vi "FRC Wizard - Robot.vi"() -> ()   [LabVIEW 2023]
uses:
  <resource>/plugins/NewDialogFiles/ProjectWizards/ProjectWizard.llb/ProjectWizard Navigation Button States.ctl
  <resource>/plugins/NewDialogFiles/ProjectWizards/ProjectWizard.llb/ProjectWizard Navigation Button State.ctl
  <resource>/plugins/NewDialogFiles/ProjectWizards/ProjectWizard.llb/ProjectWizard Navigation Buttons.ctl
  <resource>/plugins/NewDialogFiles/ProjectWizards/FRC/FRC Strings.vi
  <resource>/plugins/NewDialogFiles/ProjectWizards/FRC/frc project type.ctl
panel:
  out "project folder flag":bool
  in  "Tab Control":enum32{"Page 1"}(tab)
  in  "Framework Choice":enum32{"Robot Project"}(radio)
  in  "Team number":string="xxyy"
  out "Picture-0":picture
  in  "Project folder":path
  in  "Project name":string
  in  "Shutdown user event":refnum<user-event>
  in  "Subpanel Path user event":refnum<user-event>
  in  "Window Title user event":refnum<user-event>
  in  "Navigation Button States user event":refnum<user-event>
  in  "Navigation Buttons user event":refnum<event-registration>
  # "Select project name, folder"
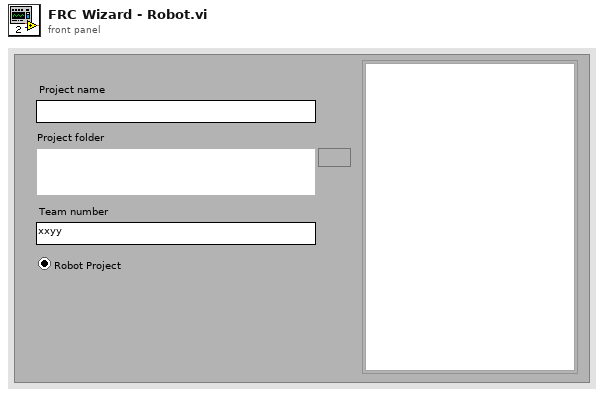
[diagram p1: front panel]
types:
  T1 = enum16{"Display", "Configure", "Hide Dialog", "Discard Ref"}
  T2 = typedef "ProjectWizard Navigation Button States.ctl" = T3[]
  T3 = typedef "ProjectWizard Navigation Button State.ctl" = cluster{"Navigation Button":T4, "Disabled":u8}
  T4 = typedef "ProjectWizard Navigation Buttons.ctl" = enum16{"Back", "Next", "Finish", "Cancel", "Help"}
  T5 = typedef "frc project type.ctl" = enum16{"arcade", "command control", "maze", "ball shooter", "dashboard", "dashboard simple", "dashboard maze", "dashboard shooter", "romi", "XRP"}
  T6 = typedef "RTNPA Navigation Buttons.ctl" = enum16{"Back", "Next", "Finish", "Cancel", "Help"}
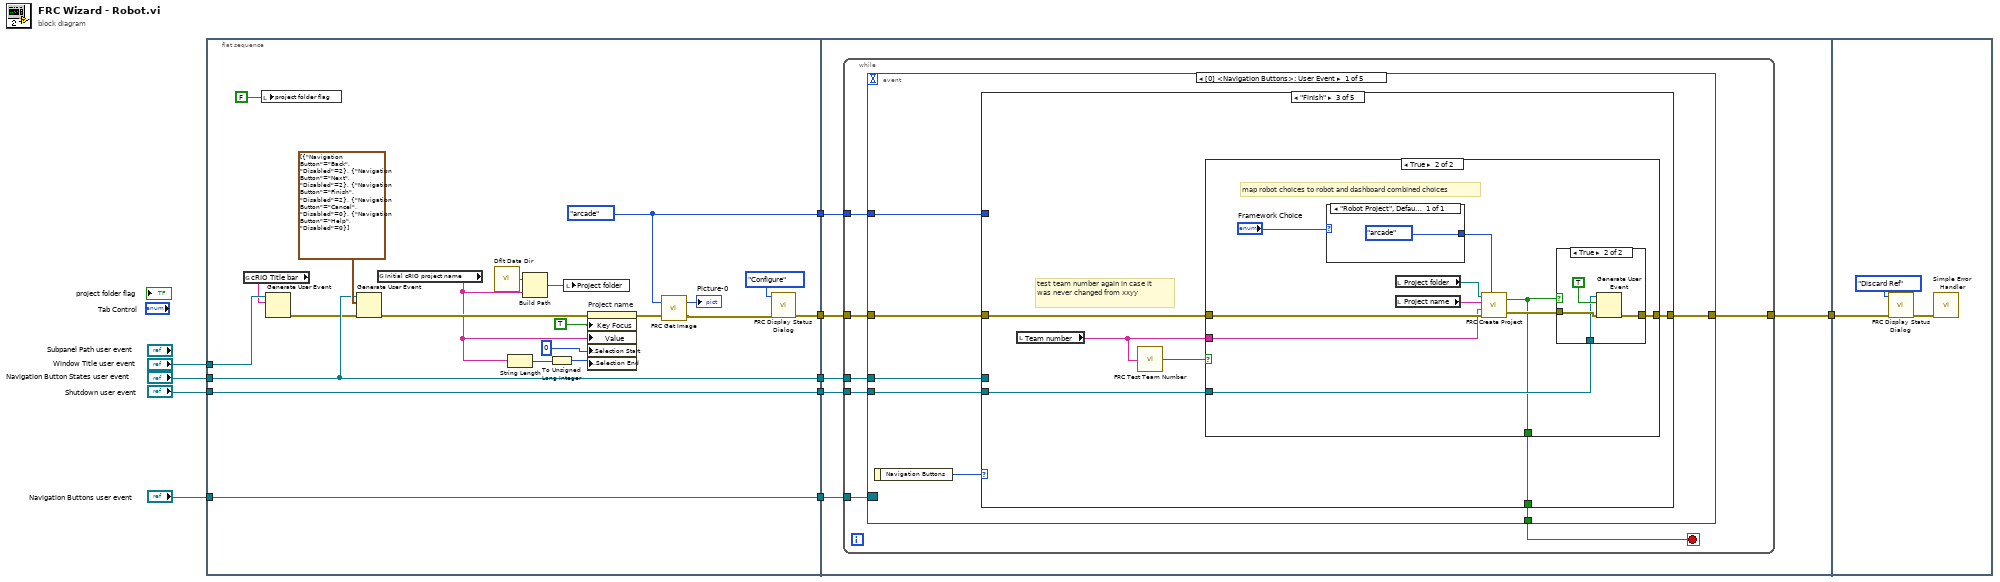
[diagram p0: block diagram]
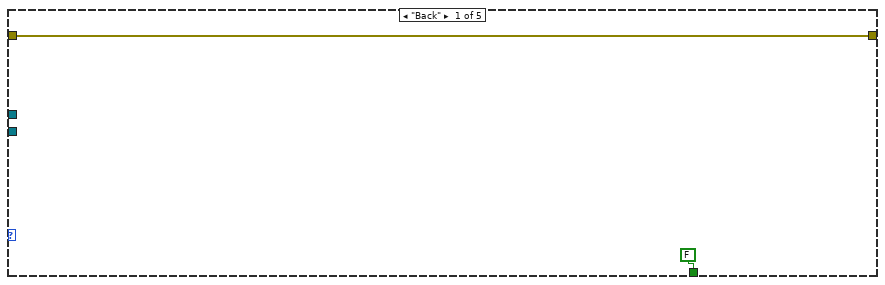
[diagram p2: hidden frame]
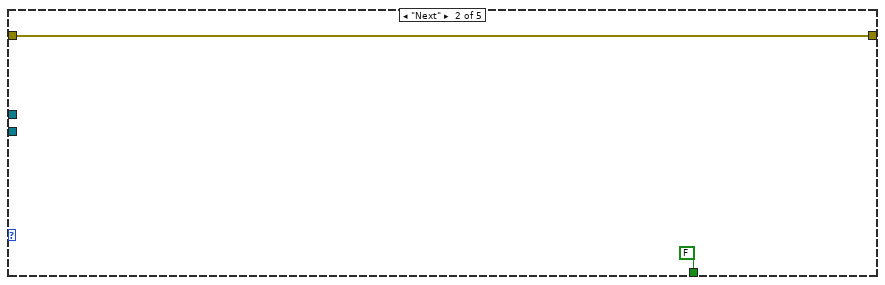
[diagram p3: hidden frame]
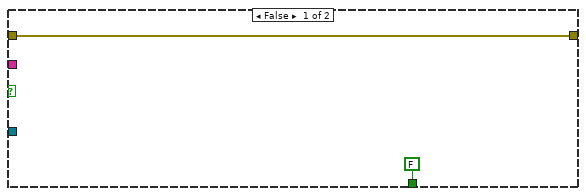
[diagram p4: hidden frame]
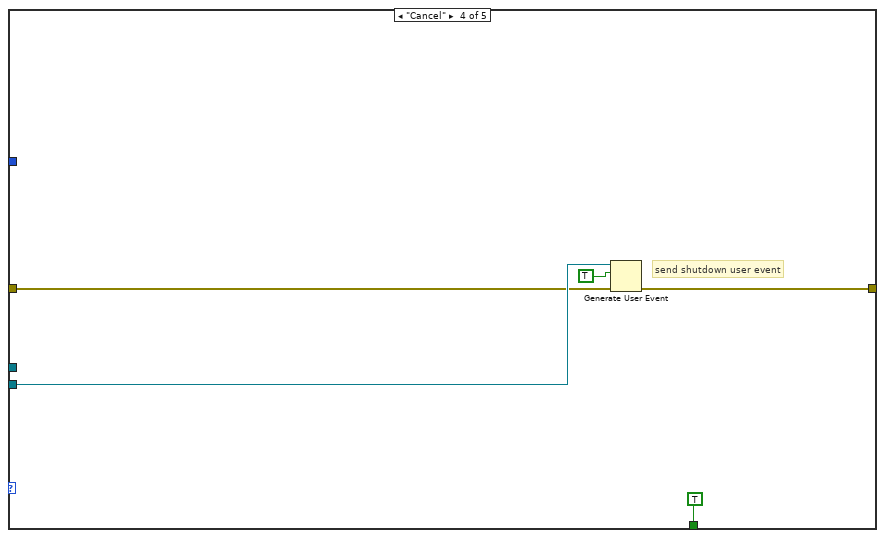
[diagram p6: hidden frame]
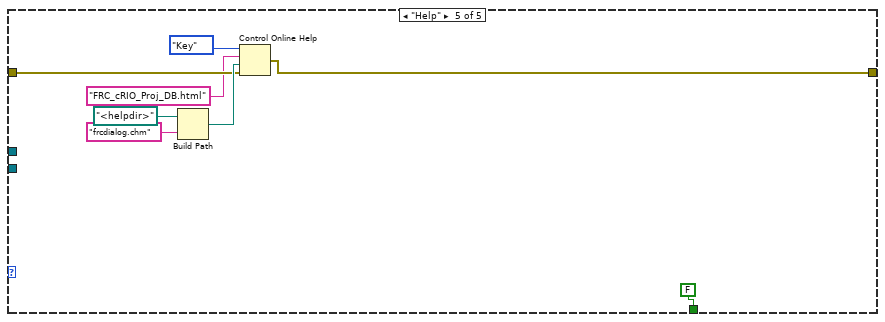
[diagram p7: hidden frame]
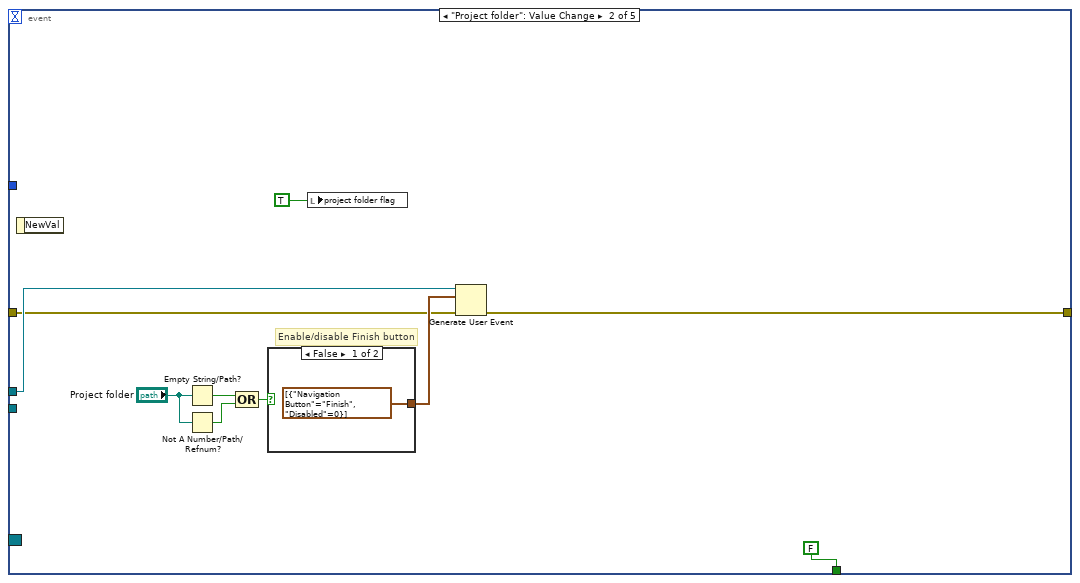
[diagram p8: hidden frame]
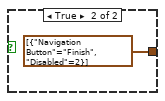
[diagram p9: hidden frame]
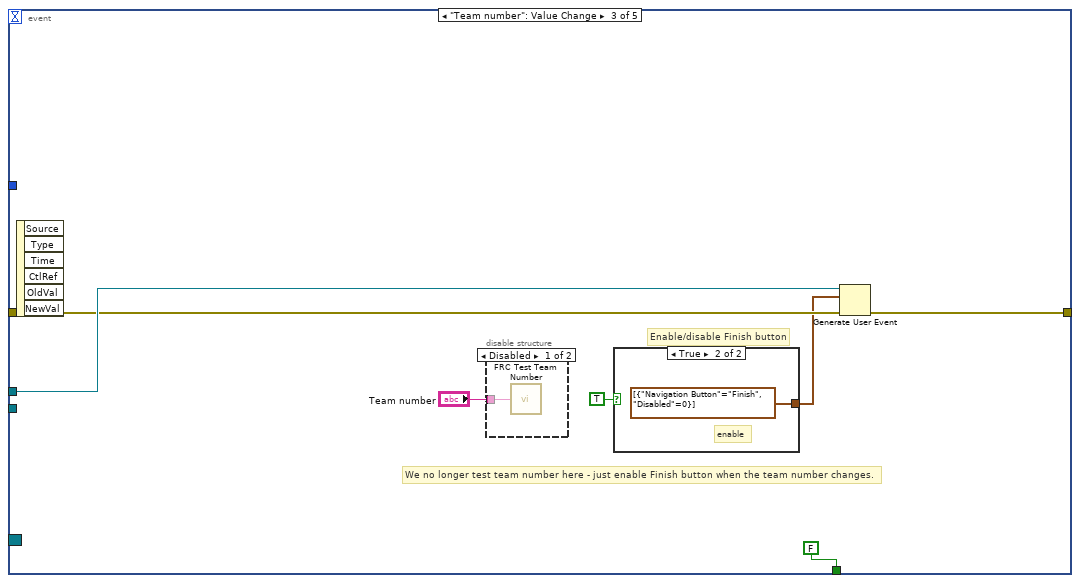
[diagram p10: hidden frame]
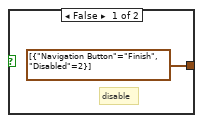
[diagram p12: hidden frame]
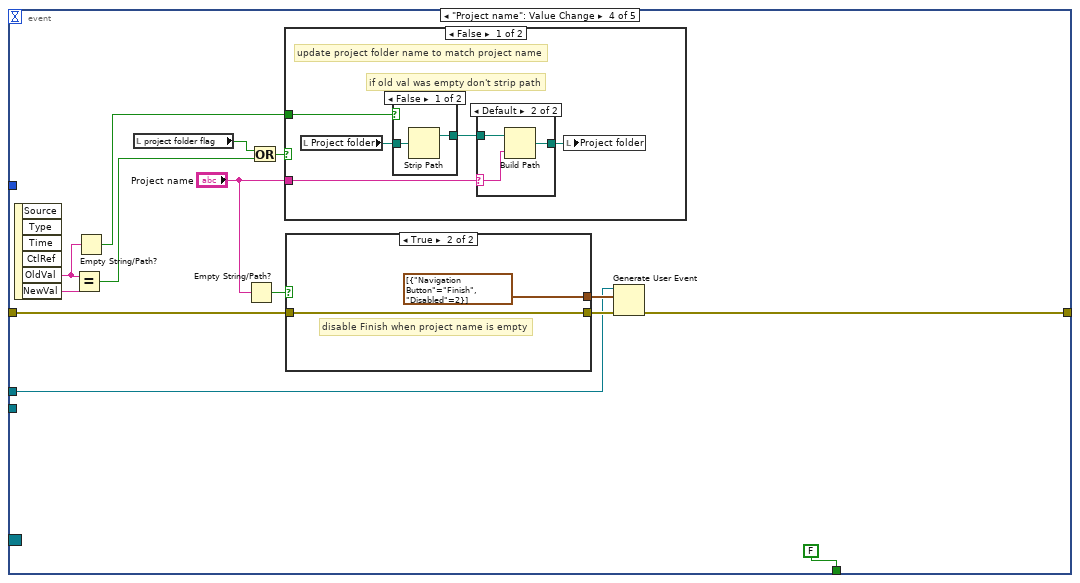
[diagram p13: hidden frame]
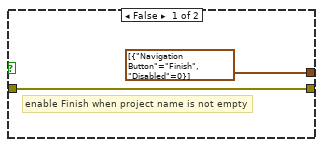
[diagram p17: hidden frame]
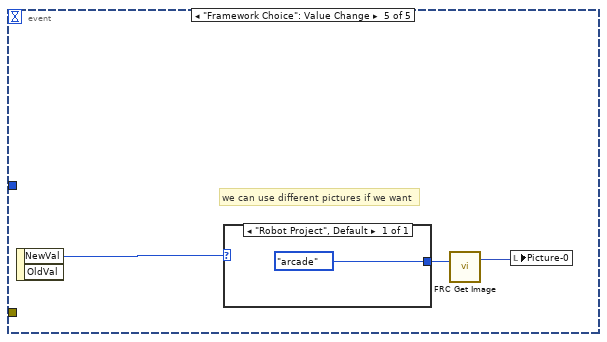
[diagram p18: hidden frame]
diagram:
  n1 = flat-sequence {
    tunnel: [w22] -> w6
    tunnel: [w32] -> w5
    tunnel: [w31] -> w4
    tunnel: [w18] -> w3
    tunnel: "Navigation Button States user event" -> [w22]
    tunnel: "Window Title user event" -> [w29]
    tunnel: "Navigation Buttons user event" -> [w32]
    tunnel: "Shutdown user event" -> [w31]
    tunnel: [w11] -> w1
    tunnel: w6 -> [w38]
    tunnel: w5 -> [w37]
    tunnel: w4 -> [w35]
    tunnel: w3 -> [w34]
    tunnel: [w36] -> w2
    tunnel: w1 -> [w33]
    tunnel: w2 -> [w151]
    frame #0 {
      w11 = frc_project_type."arcade" ("frc project type")
      n2 = global read "FRC Strings.vi" "cRIO Title bar"() -> (w26:string)
      n3 = local write "project folder flag"(FALSE ("project folder flag")) -> ()
      n4 = Generate User Event(user event=w29, event data cluster=w26) -> (error out=w21:errorcluster)  [unwired: 2 in, 1 out]
      n5 = Generate User Event(user event=w22, event data cluster=T2 [{"Navigation Button"=enum."Back", "Disabled"=2}, {"Navigation Button"=enum."Next", "Disabled"=2}, {"Navigation Button"=enum."Finish", "Disabled"=2}, {"Navigation Button"=enum."Cancel", "Disabled"=0}, {"Navigation Button"=enum."Help", "Disabled"=0}] ("Navigation Button States"), error in=w21) -> (error out=w19:errorcluster)  [unwired: 1 in, 1 out]
      n6 = global read "FRC Strings.vi" "Initial cRIO project name"() -> (w15:string)
      n7 = call <vilib>:"Dflt Data Dir.vi"() -> ("App:Default Data Directory"=w27:path)
      n8 = String Length(string=w15) -> (length=w23:i32)
      n9 = Build Path(base path=w27, name or relative path=w15) -> (appended path=w20:path)
      n10 = To Unsigned Long Integer(number=w23) -> (unsigned 32bit integer=w24:u32)
      n11 = local write "Project folder"(w20) -> ()
      n12 = property on="Project name" class="Str"(error in=w19, "Key Focus"=TRUE, "Value"=w15, "Text.Selection Start"=u32 0 ("Text.Selection:Start"), "Text.Selection End"=w24) -> (error out=w14:errorcluster)  [unwired: 1 in, 1 out]
      n13 = call <resource>:"FRC Get Image.vi"("error in"=w14, "frc project type"=w11) -> ("error out"=w13:errorcluster, "new picture"=→"Picture-0":picture)
      n14 = call <resource>:"FRC Display Status Dialog.vi"("error in"=w13, "Mode"=T1."Configure") -> ("error out"=w18:errorcluster)  [unwired: 2 in, 7 out]
    }
    frame #1 {
      n15 = while {
        tunnel: w37 -> [w45]
        tunnel: w38 -> [w44]
        tunnel: w34 -> [w43]
        tunnel: [w41] -> w36
        tunnel: w35 -> [w40]
        tunnel: w33 -> [w39]
        stop <- w42 stop-if-true
        n16 = event shown="[0] <Navigation Buttons>: User Event" {
          selector: w45 -> [_ _ _ _ _]
          dyn-events: _ -> [_ _ _ _ _]
          timeout: _ -> [_ _ _ _ _]
          tunnel: w44 -> [w48 w98 w111 w123 _]
          tunnel: w43 -> [w50 w97 w110 w128 _]
          tunnel: [w51 FALSE ("x = y?") FALSE ("x = y?") FALSE ("x = y?") _] -> w42
          tunnel: [w49 w99 w112 w125 _] -> w41
          tunnel: w40 -> [w47 _ _ _ _]
          tunnel: w39 -> [w46 _ _ _ _]
          event User Event {
            n17 = event-data() -> ("Navigation Buttons"=w52:T6)  [unwired: 1 out]
            n18 = case shown="\"Finish\"" w52 {
              tunnel: [FALSE ("x = y?") FALSE w59 TRUE FALSE] -> w51
              tunnel: w50 -> [w53 w55 w61 w81 w88]
              tunnel: [w53 w55 w62 w82 w89] -> w49
              tunnel: w48 -> [_ _ _ _ _]
              tunnel: w47 -> [_ _ w60 w83 _]
              tunnel: w46 -> [_ _ _ _ _]
              frame "Back" {
              }
              frame "Next" {
              }
              frame "Finish" {
                # "test team number again in case it was never changed from xxyy"
                n19 = local read "Team number"() -> (w58:string)
                n20 = call <resource>:"FRC Test Team Number.vi"("Team number"=w58) -> ("pass?"=w57:bool)  [unwired: 14 in]
                n21 = case shown="True" w57 {
                  tunnel: [w63 w74] -> w62
                  tunnel: w61 -> [w63 w72]
                  tunnel: w60 -> [_ w71]
                  tunnel: [FALSE ("proceed?") w68] -> w59
                  tunnel: w58 -> [_ w65]
                  frame False {
                  }
                  frame True {
                    # "map robot choices to robot and dashboard combined choices"
                    n22 = case shown="\"Robot Project\", Default" "Framework Choice" {
                      tunnel: [frc_project_type."arcade" ("frc project type")] -> w66
                      frame "Robot Project", Default {
                      }
                    }
                    n23 = local read "Project folder"() -> (w69:path)
                    n24 = local read "Project name"() -> (w70:string)
                    n25 = call <resource>:"FRC Create Project.vi"("Project folder"=w69, "Project name"=w70, "Team number"=w65, "error in"=w72, "frc project type"=w66) -> ("proceed?"=w68:bool, "error out"=w73:errorcluster)
                    n26 = case shown="True" w68 {
                      tunnel: [w76 w80] -> w74
                      tunnel: w73 -> [w76 w78]
                      tunnel: w71 -> [_ w77]
                      frame False {
                      }
                      frame True {
                        n27 = Generate User Event(user event=w77, event data cluster=TRUE ("event data"), error in=w78) -> (error out=w80:errorcluster)  [unwired: 1 in, 1 out]
                      }
                    }
                  }
                }
              }
              frame "Cancel" {
                (unwired) refnum<k0> refnum
                # "send shutdown user event"
                n28 = Generate User Event(user event=w83, event data cluster=TRUE ("event data"), error in=w81) -> (error out=w82:errorcluster)  [unwired: 1 in, 1 out]
              }
              frame "Help" {
                n29 = Build Path(base path=path "<helpdir>", name or relative path="frcdialog.chm" ("CHM or HLP filename (lvdialog.chm)")) -> (appended path=w92:path)
                n30 = Control Online Help(1:w88, 2:w92, 3:"FRC_cRIO_Proj_DB.html" ("String to search for"), 4:enum16{"Contents", "Key", "Close"}."Key" ("Operation")) -> (0:w89:errorcluster)
              }
            }
          }
          event "Project folder": Value Change {
            # "Enable/disable Finish button"
            n31 = event-data() -> ()  [unwired: 2 out]
            n32 = Empty String/Path?(string/path="Project folder") -> (empty?=w100:bool)
            n33 = Not A Number/Path/Refnum?(number/path/refnum="Project folder") -> (NaN/Path/Refnum?=w101:bool)
            n34 = Compound Arithmetic op=OR(w100, w101) -> (w102:bool)
            n35 = case shown="False" w102 {
              tunnel: [T2 [{"Navigation Button"=enum."Finish", "Disabled"=0}] ("Navigation Button States") T2 [{"Navigation Button"=enum."Finish", "Disabled"=2}] ("Navigation Button States")] -> w103
              frame False {
              }
              frame True {
              }
            }
            n36 = local write "project folder flag"(TRUE ("project folder flag")) -> ()
            n37 = Generate User Event(user event=w98, event data cluster=w103, error in=w97) -> (error out=w99:errorcluster)  [unwired: 1 in, 1 out]
          }
          event "Team number": Value Change {
            # "We no longer test team number here - just enable Finish button when the team number changes."
            # "Enable/disable Finish button"
            n38 = event-data() -> ()  [unwired: 7 out]
            n39 = disable-structure shown="Disabled" {
              disable-tunnel: "Team number" -> [w113 _]
              frame Disabled {
                n40 = call <resource>:"FRC Test Team Number.vi"("Team number"=w113) -> ()  [unwired: 14 in, 1 out]
              }
              frame Enabled {
              }
            }
            n41 = case shown="True" TRUE {
              tunnel: [T2 [{"Navigation Button"=enum."Finish", "Disabled"=2}] ("Navigation Button States") T2 [{"Navigation Button"=enum."Finish", "Disabled"=0}] ("Navigation Button States")] -> w107
              frame False {
                # "disable"
              }
              frame True {
                # "enable"
              }
            }
            n42 = Generate User Event(user event=w111, event data cluster=w107, error in=w110) -> (error out=w112:errorcluster)  [unwired: 1 in, 1 out]
          }
          event "Project name": Value Change {
            n43 = event-data() -> ("OldVal"=w117:string, "NewVal"=w121:string)  [unwired: 5 out]
            n44 = Equal?(x=w117, y=w121) -> (x = y?=w118:bool)
            n45 = Empty String/Path?(string/path=w117) -> (empty?=w116:bool)
            n46 = local read "project folder flag"() -> (w120:bool)
            n47 = Empty String/Path?(string/path="Project name") -> (empty?=w127:bool)
            n48 = Or(x=w120, y=w118) -> (x .or. y?=w119:bool)
            n49 = case shown="False" w119 {
              tunnel: "Project name" -> [w132 _]
              tunnel: w116 -> [w130 _]
              frame False {
                # "update project folder name to match project name"
                # "if old val was empty don't strip path"
                n50 = local read "Project folder"() -> (w131:path)
                n51 = case shown="False" w130 {
                  tunnel: [w136 w137] -> w133
                  tunnel: w131 -> [w135 w137]
                  frame False {
                    n52 = Strip Path(path=w135) -> (stripped path=w136:path)  [unwired: 1 out]
                  }
                  frame True {
                  }
                }
                n53 = case shown="Default" w132 {
                  selector: w132 -> [_ w139]
                  tunnel: [w138 w141] -> w134
                  tunnel: w133 -> [w138 w140]
                  frame "" {
                  }
                  frame Default {
                    n54 = Build Path(base path=w140, name or relative path=w139) -> (appended path=w141:path)
                  }
                }
                n55 = local write "Project folder"(w134) -> ()
              }
              frame True {
                # "don't update project folder, user modified it manually\nor value didn't really change"
              }
            }
            n56 = case shown="True" w127 {
              tunnel: w128 -> [w142 w144]
              tunnel: [w142 w144] -> w126
              tunnel: [T2 [{"Navigation Button"=enum."Finish", "Disabled"=0}] ("Navigation Button States") T2 [{"Navigation Button"=enum."Finish", "Disabled"=2}] ("Navigation Button States")] -> w124
              frame False {
                # "enable Finish when project name is not empty"
              }
              frame True {
                # "disable Finish when project name is empty"
              }
            }
            n57 = Generate User Event(user event=w123, event data cluster=w124, error in=w126) -> (error out=w125:errorcluster)  [unwired: 1 in, 1 out]
          }
          event "Framework Choice": Value Change {
            # "we can use different pictures if we want"
            n58 = event-data() -> ("NewVal"=w147:enum32{"Robot Project"})  [unwired: 2 out]
            n59 = case shown="\"Robot Project\", Default" w147 {
              tunnel: [frc_project_type."arcade" ("frc project type")] -> w146
              frame "Robot Project", Default {
              }
            }
            n60 = call <resource>:"FRC Get Image.vi"("frc project type"=w146) -> ("new picture"=w148:picture)  [unwired: 1 in, 1 out]
            n61 = local write "Picture-0"(w148) -> ()
          }
        }
      }
    }
    frame #2 {
      n62 = call <resource>:"FRC Display Status Dialog.vi"("error in"=w151, "Mode"=T1."Discard Ref") -> ("error out"=w150:errorcluster)  [unwired: 2 in, 7 out]
      n63 = call <vilib>:"Simple Error Handler.vi"("error in (no error)"=w150) -> ()  [unwired: 1 in, 8 out]
    }
  }
